vi "Read_Poll.vi"(5 "timeout ms":i32, 6 "pending in":u8[](array[numeric]), 7 "TLS connection":refnum<k5>, 8 "error in (no error)":errorcluster, 9 "status in":T1, 10 "frames in":T5 {"flags" format="%.0x"; "id" format="%.0x"}, 11 "rx state in":T4) -> (0 "error out":errorcluster, 1 "status out":T1, 2 "frames out":T5 {"flags" format="%.0x"; "id" format="%.0x"}, 3 "rx state out":T4, 4 "pending out":u8[](array[numeric]))   [LabVIEW 2021, in "CANsub_API.lvlib"]
doc: "API private: one Poll-mode read. State Closed ? 5202, Lost ? 5203 (count 0). Open: TCP Read (Immediate, 4096 B, timeout ms) ? pending (leftover, first call only) ? C_Decode_To_Frames into the caller’s frames ? pong (W7) if a ping arrived ? counters. TCP/decode/pong error or peer close ? state = Lost, error 5203. Loop-safe: no allocation, bounded time (except LabVIEW’s TCP Read/Write strings)."
uses:
  CANsub_API.lvlib
  Typedefs/CANsub_State.ctl
  C_RX_State.ctl
  CANsub_C.lvlib
  Typedefs/CANsub_Frames.ctl
  common/Typedefs/Bit_Timing.ctl
  common/CANsub_Common.lvlib
  Typedefs/CANsub_Status.ctl
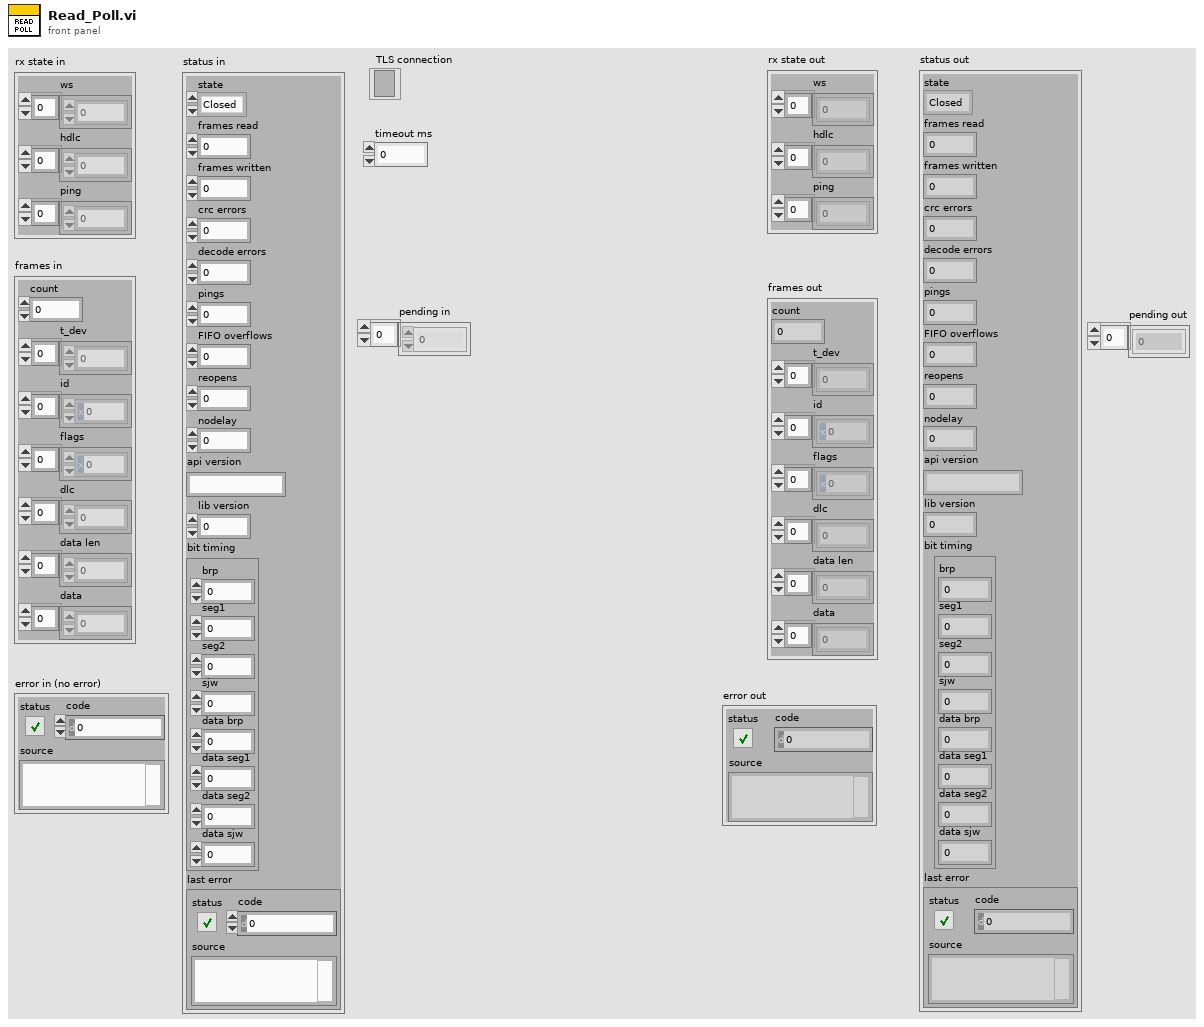
[diagram p1: front panel]
types:
  T1 = typedef "CANsub_API.lvlib/CANsub_Status.ctl" = cluster{"state":T2, "frames read":u32, "frames written":u32, "crc errors":u32, "decode errors":i32, "pings":u32, "FIFO overflows":u32, "reopens":u32, "nodelay":i32, "api version":string, "lib version":u32, "bit timing":T3, "last error":errorcluster}
  T2 = typedef "CANsub_API.lvlib/CANsub_State.ctl" = enum16{"Closed", "Open", "Lost"}
  T3 = typedef "CANsub_Common.lvlib/Bit_Timing.ctl" = cluster{"brp":u16, "seg1":u16, "seg2":u16, "sjw":u16, "data brp":u16, "data seg1":u16, "data seg2":u16, "data sjw":u16}
  T4 = typedef "CANsub_C.lvlib/C_RX_State.ctl" = cluster{"ws":u8[], "hdlc":u8[], "ping":u8[]}
  T5 = typedef "CANsub_API.lvlib/CANsub_Frames.ctl" = cluster{"count":i32, "t_dev":dbl[], "id":u32[], "flags":u16[], "dlc":u8[], "data len":u8[], "data":u8[]}
  T6 = enum16{"Standard", "Buffered", "CRLF", "Immediate"}
  T7 = typedef "CANsub_C.lvlib/C_Decode_Result.ctl" = cluster{"n frames":i32, "peer close":bool, "ping len":i32, "crc errors":u32, "decode errors":i32}
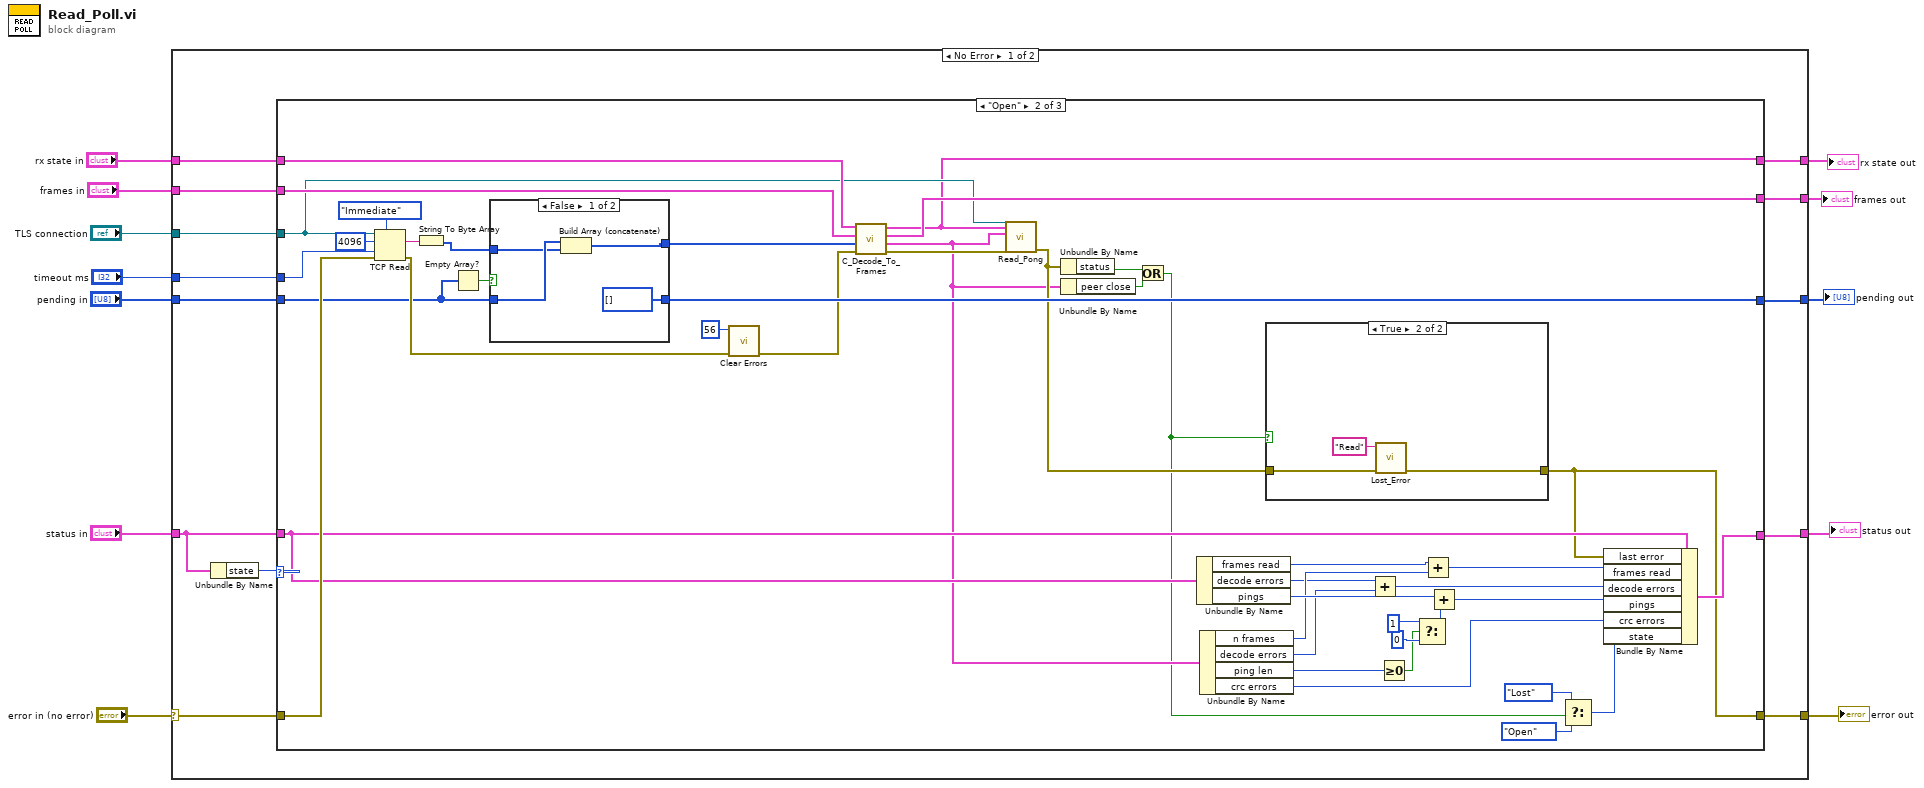
[diagram p0: block diagram]
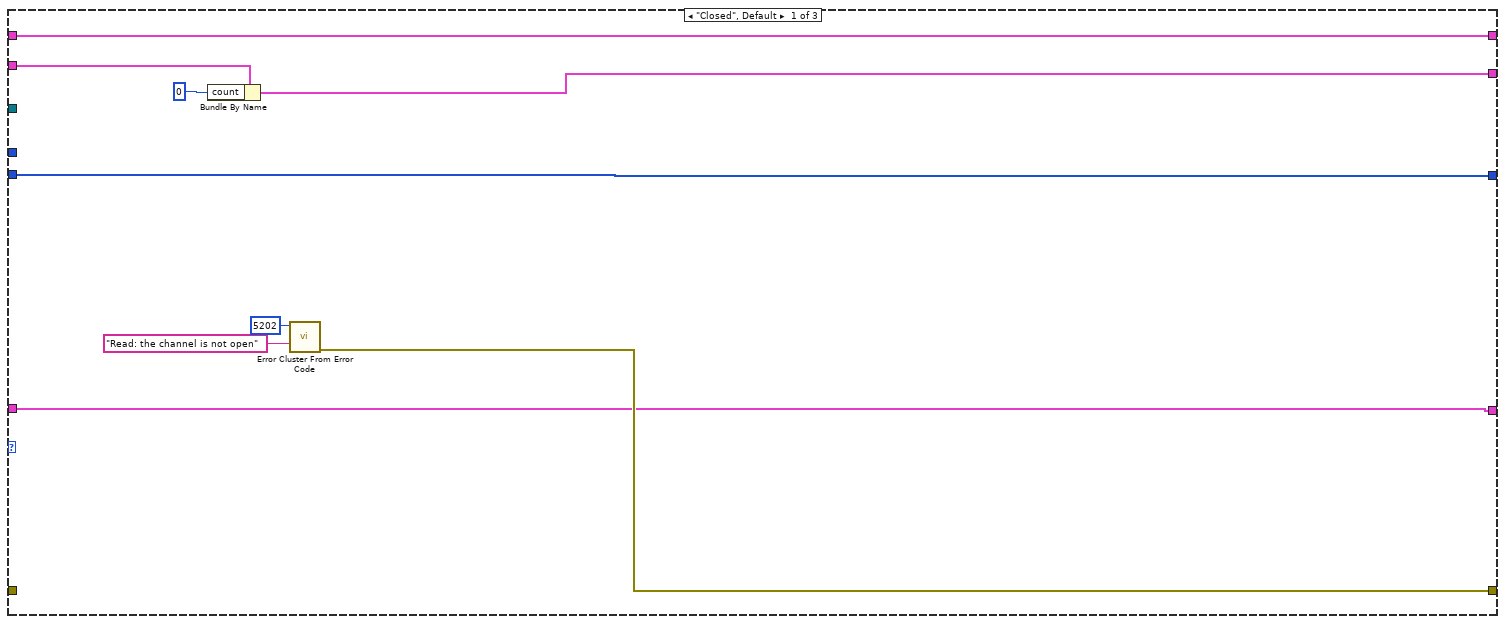
[diagram p2: hidden frame]
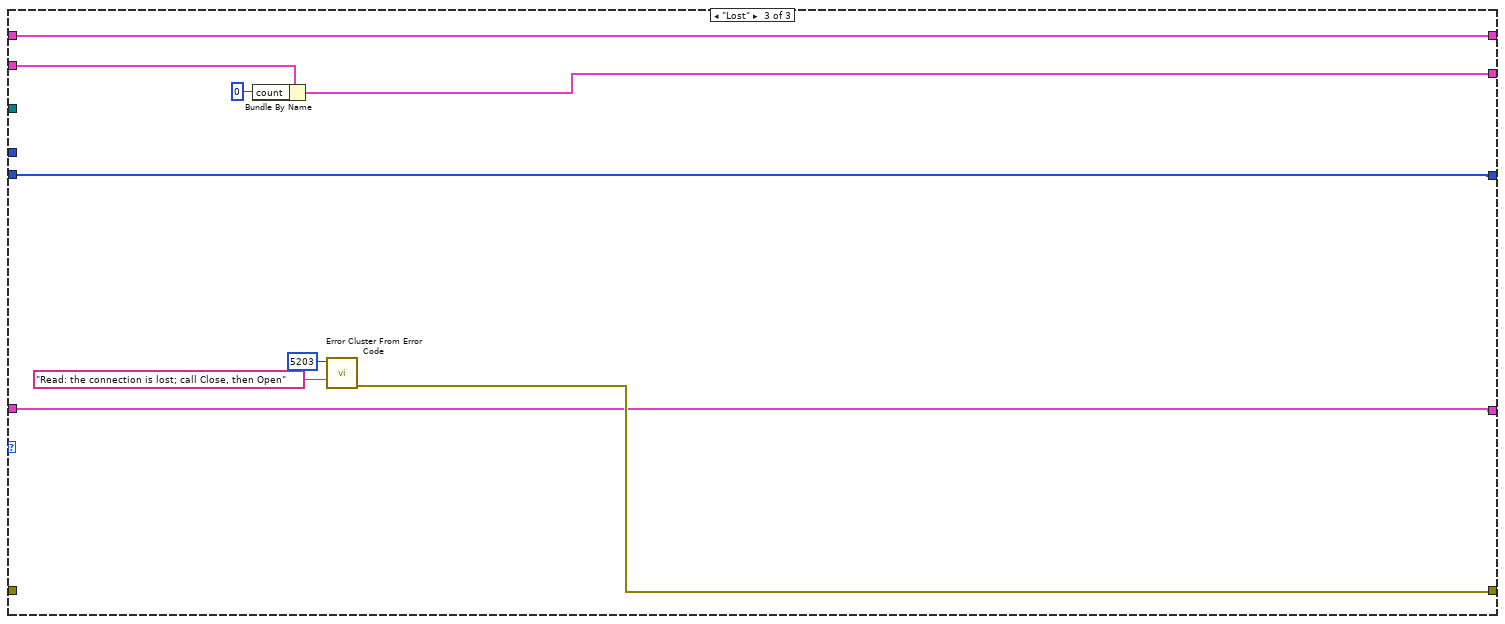
[diagram p5: hidden frame]
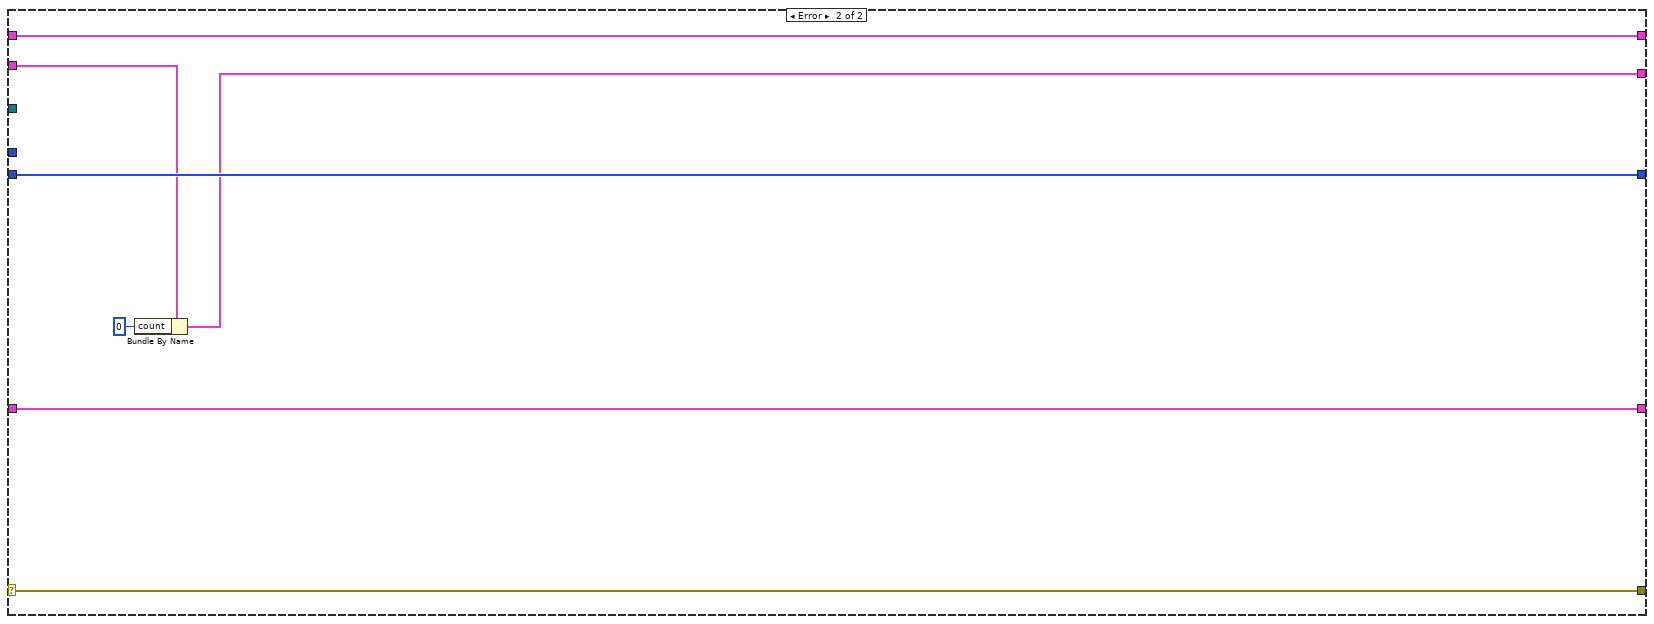
[diagram p6: hidden frame]
diagram:
  n1 = case shown="No Error" "error in (no error)" {
    selector: "error in (no error)" -> [w16 w98]
    tunnel: [w19 w104] -> w11
    tunnel: "rx state in" -> [w18 w104]
    tunnel: [w21 w103] -> w9
    tunnel: "pending in" -> [w20 w103]
    tunnel: "frames in" -> [w23 w102]
    tunnel: [w22 w100] -> w6
    tunnel: [w13 w99] -> w5
    tunnel: "status in" -> [w14 w99]
    tunnel: [w24 w98] -> w3
    tunnel: "TLS connection" -> [w17 _]
    tunnel: "timeout ms" -> [w15 _]
    frame No Error {
      n2 = Unbundle By Name(w14) -> ("state"=w25:T2)
      n3 = case shown="\"Open\"" w25 {
        tunnel: [w32 w38 w90] -> w24
        tunnel: w23 -> [w31 w67 w94]
        tunnel: [w29 w66 w93] -> w22
        tunnel: [w28 w72 w92] -> w21
        tunnel: w20 -> [w28 w35 w92]
        tunnel: [w27 w62 w91] -> w19
        tunnel: w18 -> [w27 w69 w91]
        tunnel: w17 -> [_ w65 _]
        tunnel: w16 -> [_ w76 _]
        tunnel: w15 -> [_ w74 _]
        tunnel: w14 -> [w26 w59 w89]
        tunnel: [w26 w58 w89] -> w13
        frame "Closed", Default {
          n4 = Bundle By Name(cluster=w31, "count"=0) -> (w29:T5)
          n5 = call <vilib>:"Error Cluster From Error Code.vi"("error message (\"\")"="Read: the channel is not open" ("error message (\"\")"), "error code (0)"=5202) -> ("error out"=w32:errorcluster)  [unwired: 7 in]
        }
        frame "Open" {
          n6 = TCP Read(connection ID=w65, bytes to read=4096, error in (no error)=w76, 7:T6."Immediate" ("mode (standard)"), 9:w74) -> (data out=w73:string, error out=w68:errorcluster)  [unwired: 1 out]
          n7 = String To Byte Array(string=w73) -> (unsigned byte array=w71:u8[])
          n8 = Empty Array?(array=w35) -> (empty?=w77:bool)
          n9 = case shown="False" w77 {
            tunnel: [u8[] [] ("pending in") w88] -> w72
            tunnel: w35 -> [w86 w88]
            tunnel: w71 -> [w85 w87]
            tunnel: [w84 w87] -> w70
            frame False {
              n10 = Build Array (concatenate)(w86, w85) -> (w84:u8[])
            }
            frame True {
            }
          }
          n11 = call <vilib>:"Clear Errors.vi"("error in (no error)"=w68, "specific error code to clear (0: all)"=56) -> ("error out"=w37:errorcluster)  [unwired: 4 in, 1 out]
          n12 = call "C_Decode_To_Frames.vi"("error in (no error)"=w37, "bytes in"=w70, "frames in"=w67, "state in"=w69) -> ("error out"=w64:errorcluster, "result"=w57:T7, "frames out"=w66:T5, "state out"=w62:T4)  [unwired: 4 in]
          n13 = call "Read_Pong.vi"("error in (no error)"=w64, "rx state"=w62, "result"=w57, "TLS connection"=w65) -> ("error out"=w60:errorcluster)  [unwired: 7 in]
          n14 = Unbundle By Name(w60) -> ("status"=w63:bool)
          n15 = Unbundle By Name(w57) -> ("peer close"=w61:bool)
          n16 = Or(x=w63, y=w61) -> (x .or. y?=w56:bool)
          n17 = Unbundle By Name(w59) -> ("frames read"=w43:u32, "decode errors"=w41:i32, "pings"=w52:u32)
          n18 = Unbundle By Name(w57) -> ("n frames"=w44:i32, "decode errors"=w40:i32, "ping len"=w49:i32, "crc errors"=w45:u32)
          n19 = case shown="True" w56 {
            tunnel: w60 -> [w79 w81]
            tunnel: [w79 w80] -> w38
            frame False {
            }
            frame True {
              n20 = call "Lost_Error.vi"("cause"=w81, "operation"="Read") -> ("error out"=w80:errorcluster)  [unwired: 9 in]
            }
          }
          n21 = Add(x=w41, y=w40) -> (x+y=w39:i32)
          n22 = Greater Or Equal To 0?(x=w49) -> (x >= 0?=w48:bool)
          n23 = Select(t=u32 1, s=w48, f=u32 0) -> (s? t:f=w47:u32)
          n24 = Add(x=w43, y=w44) -> (x+y=w42:u32)
          n25 = Add(x=w52, y=w47) -> (x+y=w46:u32)
          n26 = Select(t=CANsub_State."Lost" ("state"), s=w56, f=CANsub_State."Open" ("state")) -> (s? t:f=w53:T2)
          n27 = Bundle By Name(cluster=w59, "last error"=w38, "frames read"=w42, "decode errors"=w39, "pings"=w46, "crc errors"=w45, "state"=w53) -> (w58:T1)
        }
        frame "Lost" {
          n28 = Bundle By Name(cluster=w94, "count"=0) -> (w93:T5)
          n29 = call <vilib>:"Error Cluster From Error Code.vi"("error message (\"\")"="Read: the connection is lost; call Close, then Open" ("error message (\"\")"), "error code (0)"=5203) -> ("error out"=w90:errorcluster)  [unwired: 7 in]
        }
      }
    }
    frame Error {
      n30 = Bundle By Name(cluster=w102, "count"=0) -> (w100:T5)
    }
  }
  "error out" <- w3
  "frames out" <- w6
  "rx state out" <- w11
  "pending out" <- w9
  "status out" <- w5
